vi "EditOptions.vi"(8 "error in":errorcluster, 11 "Module Editor Node in":refnum<class "module editor node.lvclass">) -> (0 "error out":errorcluster, 1 "edit options":T1, 2 "subnodes class":T2, 3 "Module Editor Node out":refnum<class "module editor node.lvclass">)   [LabVIEW 2013, in "PL Framework Configuration Tool.lvlib" / "module editor node.lvclass"]
doc: "This VI Contains the options for the Menu that will be displayed when doing right click on an item\nThe subnodes class configures which nodes can be added to this nodes\nAnd the edit options determine which options are available for the node.\n\nThis configuration is stored in this VI in case some dynamic configuration is required for the menu options or subnodes.\n\nAll VIs must overide this method"
uses:
  module editor node.lvclass
  <vilib>/NI/Configuration Framework/Node/SubNodeCluster.ctl
  <vilib>/NI/Configuration Framework/Node/NodeMenuOptions.ctl
  <vilib>/NI/Configuration Framework/serializable configuration/NISE_CEF_serializable configuration.lvclass
  <vilib>/NI/Configuration Framework/Node/NISE_CEF_Node.lvclass
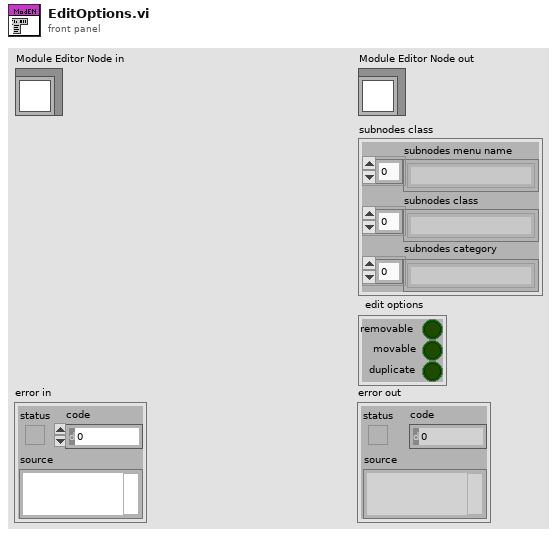
[diagram p1: front panel]
types:
  T1 = typedef "NISE_CEF_Node.lvclass/NodeMenuOptions.ctl" = cluster{"removable":bool, "movable":bool, "duplicate":bool}
  T2 = typedef "NISE_CEF_Node.lvclass/SubNodeCluster.ctl" = cluster{"subnodes menu name":string[], "subnodes class":string[], "subnodes category":string[]}
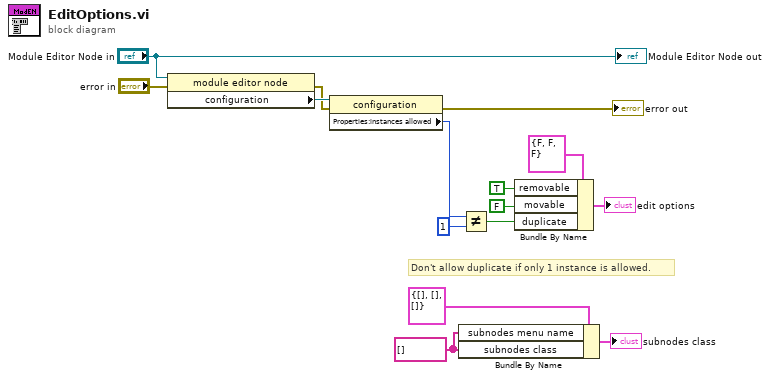
[diagram p0: block diagram]
diagram:
  w11 = string[] [] ("subnodes menu name")
  # "Don't allow duplicate if only 1 instance is allowed."
  n1 = property class="module editor node"(reference="Module Editor Node in", error in="error in") -> (error out=w5:errorcluster, "configuration"=w7:refnum<class "NISE_CEF_serializable configuration.lvclass">)  [unwired: 1 out]
  n2 = property class="configuration"(reference=w7, error in=w5) -> (error out=→"error out":errorcluster, "Properties:instances allowed"=w3:i32)  [unwired: 1 out]
  n3 = Bundle By Name(cluster=T2 {"subnodes menu name"=[], "subnodes class"=[], "subnodes category"=[]} ("subnodes class"), "subnodes menu name"=w11, "subnodes class"=w11) -> (→"subnodes class":T2)
  n4 = Not Equal?(x=w3, y=1) -> (x != y?=w1:bool)
  n5 = Bundle By Name(cluster=T1 {"removable"=FALSE, "movable"=FALSE, "duplicate"=FALSE} ("edit options"), "removable"=TRUE, "movable"=FALSE, "duplicate"=w1) -> (→"edit options":T1)
  "Module Editor Node out" <- "Module Editor Node in"
